vi "Frame Configuration Page.vi"(8 "error in (no error)":errorcluster, 11 "Node Ptr":T2 format="%.0x") -> (0 "error out":errorcluster)   [LabVIEW 2015, in "Protection and Rolling Counter Addon System Explorer.lvlib"]
uses:
  Protection and Rolling Counter Addon System Explorer.lvlib
  <vilib>/NI Veristand/Custom Device API/Custom Device Item Ref.ctl
  Shared/Types/Protection Type.ctl
  <vilib>/NI Veristand/Custom Device API/Custom Device API.lvlib
  Shared/Protection and Rolling Counter Addon Shared.lvlib
panel:
  in  "Protection Type":T1
  out "Frame ID":u32 format="%.0x"
  in  "Max Count":dbl=4.0
  out "Frame Rate":dbl
  out "Rolling Counter Channel":string
  out "CRC Channel":string
  in  "SHDocVw.IWebBrowser":refnum<k7>(container)
  in  "Value":dbl
  in  "Monitored Channels":i32(listbox)
  in  "Header":cluster{"Section Name":string}={"Section Name"="Custom Device Item Settings"}
  in  "Description":string
  in  "Name":string
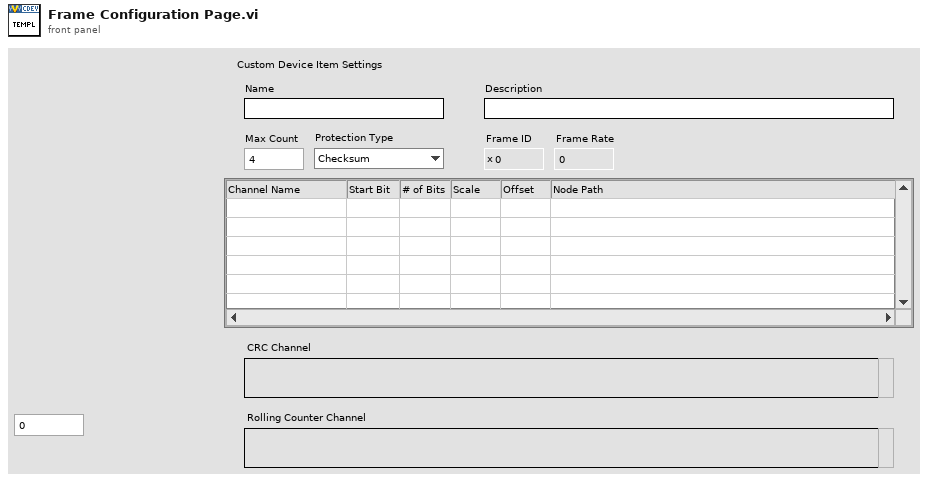
[diagram p1: front panel]
types:
  T1 = typedef "Protection and Rolling Counter Addon Shared.lvlib/Protection Type.ctl" = enum16{"Checksum", "CRC", "None (Counter Only)"}
  T2 = typedef "Custom Device API.lvlib/Custom Device Item Ref.ctl" = u64
  T3 = typedef "Custom Device API.lvlib/Custom Device Item Info.ctl" = cluster{"Name":string, "Is Channel":bool, "GUID":string, "Is Waveform":bool}
  T4 = typedef "Protection and Rolling Counter Addon Shared.lvlib/FrameConfiguration.ctl" = cluster{"Input Channels":T5[], "Frame Rate":dbl, "Rolling Counter Count":dbl, "PCL Count":u64, "Max Count":dbl, "Frame ID":u32, "Rolling Counter":T5, "CRC":T5, "Frame Name":string, "Cluster":string, "Database":string, "Protection Type":T1}
  T5 = typedef "Protection and Rolling Counter Addon Shared.lvlib/InputChannelConfiguration.ctl" = cluster{"Start Bit":i32, "Name":string, "Node Path":string, "Number of bits":i32, "Scale":dbl, "Offset":dbl, "Data Type":u32}
  T6 = typedef "Custom Device API.lvlib/Custom Device Commands.ctl" = enum16{"Default", "Item renamed", "Shutdown", "Dynamic button pressed"}
  T7 = typedef "LVPoint32TypeDef.ctl" = cluster{"Horizontal":i32, "Vertical":i32}
  T8 = typedef "LVRowAndColumnTypeDef.ctl" = cluster{"Row":i32, "Column":i32}
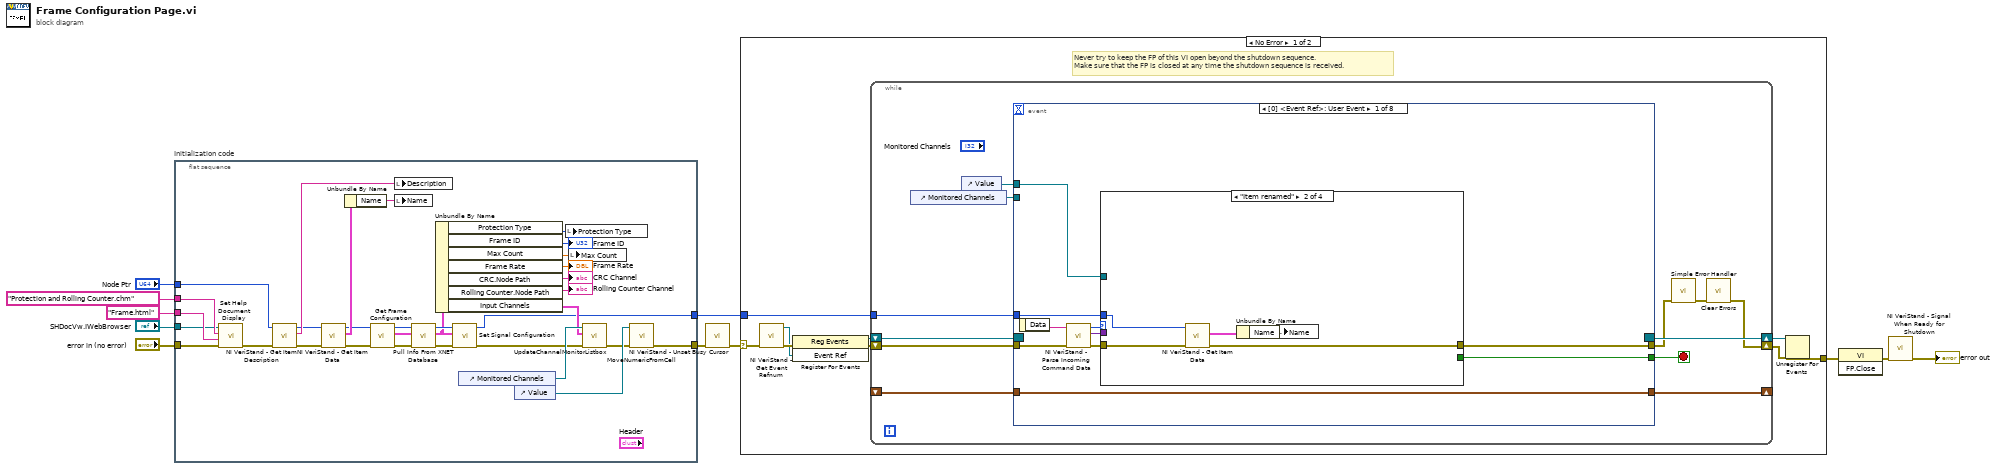
[diagram p0: block diagram]
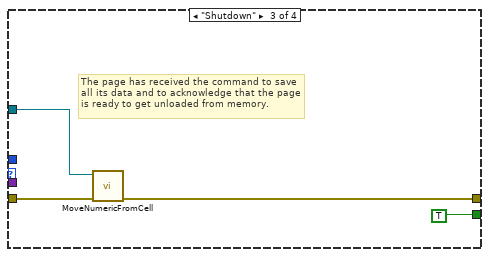
[diagram p3: hidden frame]
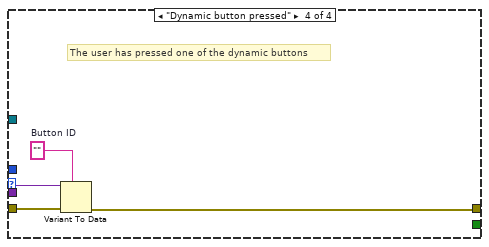
[diagram p4: hidden frame]
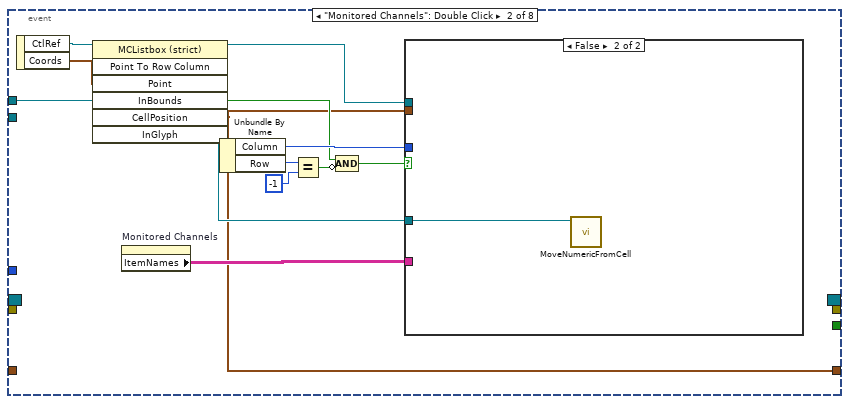
[diagram p5: hidden frame]
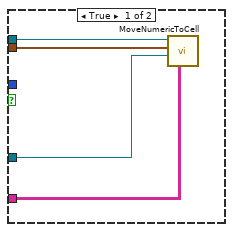
[diagram p6: hidden frame]
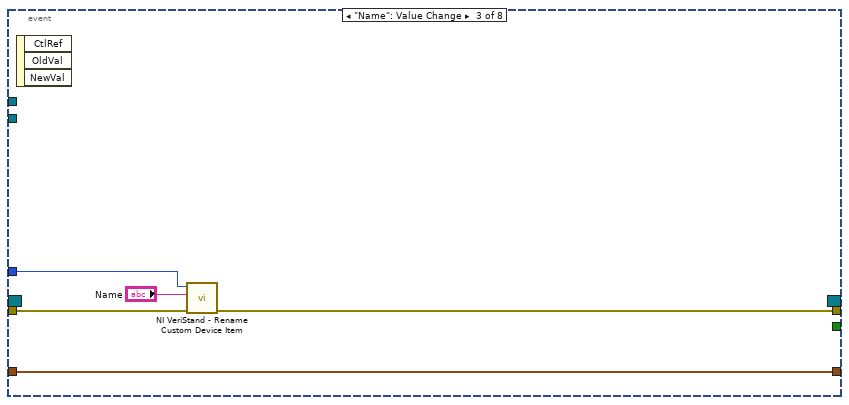
[diagram p7: hidden frame]
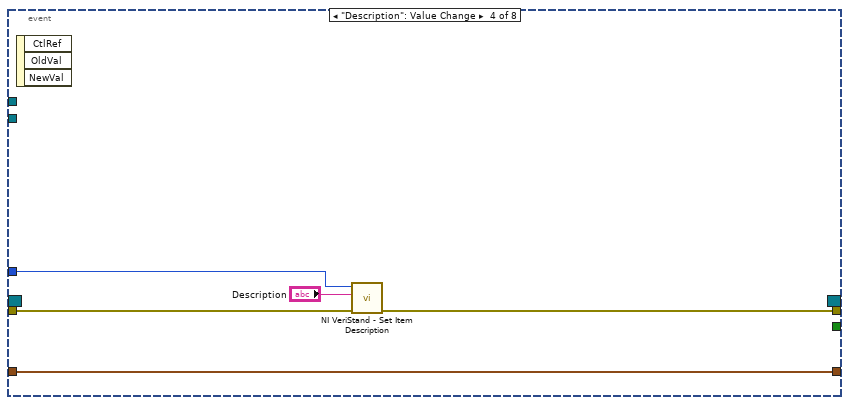
[diagram p8: hidden frame]
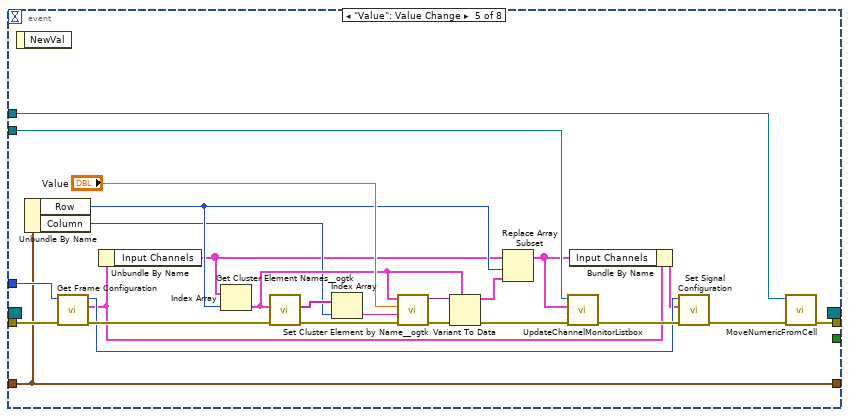
[diagram p9: hidden frame]
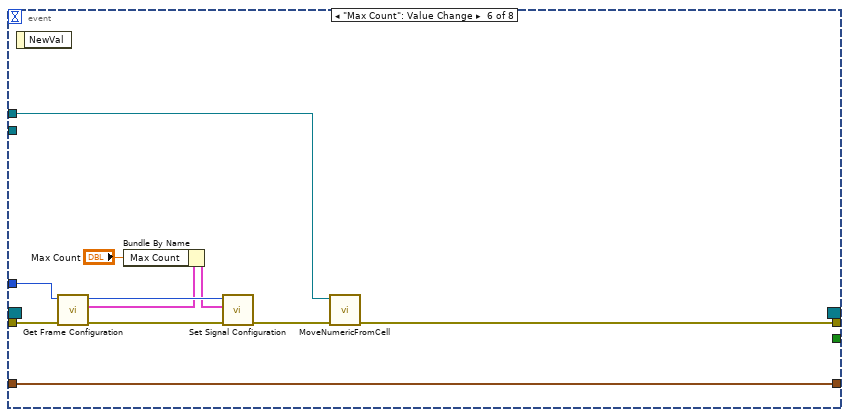
[diagram p10: hidden frame]
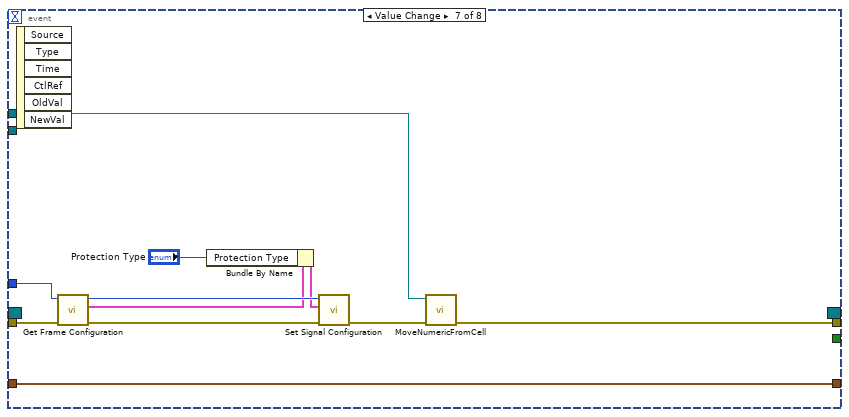
[diagram p11: hidden frame]
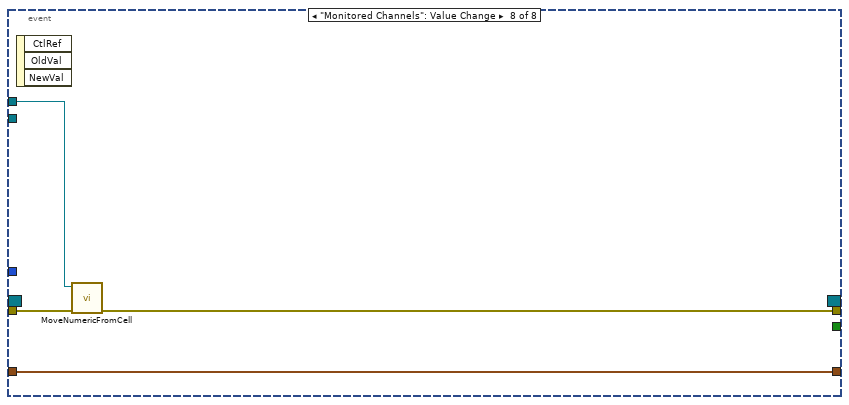
[diagram p12: hidden frame]
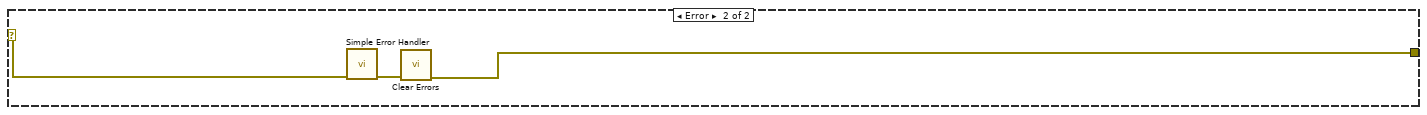
[diagram p13: hidden frame]
diagram:
  n1 = flat-sequence "Initialization code" {
    tunnel: "error in (no error)" -> [w39]
    tunnel: "Node Ptr" -> [w28]
    tunnel: [w36] -> w9
    tunnel: [w13] -> w7
    tunnel: "Protection and Rolling Counter.chm" ("Main CHM File") -> [w43]
    tunnel: "Frame.html" ("HTML File") -> [w42]
    tunnel: "SHDocVw.IWebBrowser" -> [w41]
    frame #0 {
      n2 = call "Set Help Document Display.vi"("error in (no error)"=w39, "HTML File"=w42, "Main CHM File"=w43, "SHDocVw.IWebBrowser2"=w41) -> ("error out"=w29:errorcluster)  [unwired: 7 in]
      n3 = call <vilib>:"NI VeriStand - Get Item Description.vi"("error in (no error)"=w29, "Item Ref in"=w28) -> ("error out"=w32:errorcluster, "Description"=w31:string, "Item Ref out"=w30:T2)  [unwired: 7 out]
      n4 = call <vilib>:"NI VeriStand - Get Item Data.vi"("error in (no error)"=w32, "Item Ref in"=w30) -> ("error out"=w19:errorcluster, "Item Info"=w33:T3, "Item Ref out"=w18:T2)  [unwired: 7 out]
      n5 = Unbundle By Name(w33) -> ("Name"=w34:string)
      n6 = call "Get Frame Configuration.vi"("error in"=w19, "Parent Ref"=w18) -> ("error out"=w20:errorcluster, "Selected Channels"=w16:T4, "Parent Ref Out"=w17:T2)  [unwired: 7 in]
      n7 = local write "Description"(w31) -> ()
      n8 = local write "Name"(w34) -> ()
      n9 = call "Pull Info From XNET Database.vi"("error in"=w20, "Frame Configuration"=w16, "Parent Ref"=w17) -> ("error out"=w21:errorcluster, "Frame Configuration"=w14:T4, "Item Ref out"=w15:T2)  [unwired: 6 in]
      n10 = Unbundle By Name(w14) -> ("Protection Type"=w22:T1, "Frame ID"=→"Frame ID":u32, "Max Count"=w24:dbl, "Frame Rate"=→"Frame Rate":dbl, "CRC.Node Path"=→"CRC Channel":string, "Rolling Counter.Node Path"=→"Rolling Counter Channel":string, "Input Channels"=w35:T5[])
      n11 = call "Set Signal Configuration.vi"("error in"=w21, "Selected Channels"=w14, "Parent Ref"=w15) -> ("error out"=w12:errorcluster, "Parent Ref Out"=w13:T2)  [unwired: 7 in]
      n12 = control-ref of="Monitored Channels"() -> (w40:refnum<vi>)
      n13 = control-ref of="Value"() -> (w38:refnum<vi>)
      n14 = local write "Protection Type"(w22) -> ()
      n15 = local write "Max Count"(w24) -> ()
      n16 = call "UpdateChannelMonitorListbox.vi"("error in (no error)"=w12, "Monitored Channels"=w35, "Listbox"=w40) -> ("error out"=w37:errorcluster)  [unwired: 8 in]
      n17 = call "MoveNumericFromCell.vi"("error in (no error)"=w37, "Digital in"=w38) -> ("error out"=w36:errorcluster)  [unwired: 9 in]
    }
  }
  n18 = call <vilib>:"NI VeriStand - Unset Busy Cursor.vi"("error in (no error)"=w9) -> ("error out"=w8:errorcluster)  [unwired: 10 out]
  n19 = case shown="No Error" w8 {
    selector: w8 -> [w44 w169]
    tunnel: [w49 w167] -> w11
    tunnel: w7 -> [w45 _]
    frame No Error {
      # "Never try to keep the FP of this VI open beyond the shutdown sequence.\nMake sure that the FP is closed at any time the shutdown sequence is received."
      n20 = call <vilib>:"NI VeriStand - Get Event Refnum.vi"("error in (no error)"=w44) -> ("error out"=w52:errorcluster, "Event Ref"=w48:refnum<user-event>)  [unwired: 9 out]
      n21 = register-events(error in=w52, w48) -> (reference out=w46:refnum<event-registration>, error out=w47:errorcluster)  [unwired: 1 in]
      n22 = while {
        tunnel: w45 -> [w60]
        shift-right: [w57] -> w50
        shift-left: w47 -> [w63]
        shift-right: [w64] -> w51
        shift-left: w46 -> [w62]
        shift-right: [w55] -> _
        shift-left: _ -> [w54]
        stop <- w61 stop-if-true
        n23 = control-ref of="Monitored Channels"() -> (w53:refnum<vi>)
        n24 = control-ref of="Value"() -> (w56:refnum<vi>)
        n25 = event shown="[0] <Event Ref>: User Event" {
          selector: w62 -> [_ _ _ _ _ _ _ _]
          dyn-events: [_ _ _ _ _ _ _ _] -> w64
          timeout: _ -> [_ _ _ _ _ _ _ _]
          tunnel: w63 -> [w74 _ w108 w113 w138 w149 w160 w164]
          tunnel: [w70 _ _ _ _ _ _ _] -> w61
          tunnel: [w69 _ w106 w112 w122 w146 w157 w163] -> w59
          tunnel: w60 -> [w68 _ w107 w111 w139 w150 w161 _]
          tunnel: w56 -> [w65 w96 _ _ w140 w151 w162 w165]
          tunnel: [w66 w89 w110 w115 w134 w147 w158 w166] -> w55
          tunnel: w54 -> [w66 _ w110 w115 w134 w147 w158 w166]
          tunnel: w53 -> [_ _ _ _ w137 _ _ _]
          event User Event {
            n26 = event-data() -> ("Data"=w73:string)  [unwired: 1 out]
            n27 = call <vilib>:"NI VeriStand - Parse Incoming Command Data.vi"("error in (no error)"=w74, "Incoming data"=w73) -> ("error out"=w72:errorcluster, "Outgoing data"=w67:variant, "Action"=w71:T6)  [unwired: 7 out]
            n28 = case shown="\"Item renamed\"" w71 {
              tunnel: w72 -> [w75 w78 w82 w88]
              tunnel: [_ _ TRUE _] -> w70
              tunnel: [w75 w77 w81 w85] -> w69
              tunnel: w68 -> [_ w76 _ _]
              tunnel: w67 -> [_ _ _ w87]
              tunnel: w65 -> [_ _ w83 _]
              frame "Default", Default {
              }
              frame "Item renamed" {
                n29 = call <vilib>:"NI VeriStand - Get Item Data.vi"("error in (no error)"=w78, "Item Ref in"=w76) -> ("error out"=w77:errorcluster, "Item Info"=w79:T3)  [unwired: 8 out]
                n30 = Unbundle By Name(w79) -> ("Name"=w80:string)
                n31 = local write "Name"(w80) -> ()
              }
              frame "Shutdown" {
                # "The page has received the command to save all its data and to acknowledge that the page is ready to get unloaded from memory."
                n32 = call "MoveNumericFromCell.vi"("error in (no error)"=w82, "Digital in"=w83) -> ("error out"=w81:errorcluster)  [unwired: 9 in]
              }
              frame "Dynamic button pressed" {
                w86 = ""  # Button ID
                # "The user has pressed one of the dynamic buttons"
                n33 = Variant To Data(error in=w88, type=w86, Variant=w87) -> (error out=w85:errorcluster)  [unwired: 1 out]
              }
            }
          }
          event "Monitored Channels": Double Click {
            n34 = event-data() -> ("CtlRef"=w99:refnum<vi>, "Coords"=w98:T7)  [unwired: 1 out]
            n35 = invoke class="MCListbox (strict)" method="Point To Row Column"(reference=w99, "Point"=w98) -> (reference out=w97:refnum<vi>, "InBounds"=w93:bool, "CellPosition"=w89:T8)  [unwired: 5 in, 4 out]
            n36 = property on="Monitored Channels" class="MCListbox (strict)"() -> ("ItemNames"=w90:string[][])  [unwired: 2 in, 2 out]
            n37 = Unbundle By Name(w89) -> ("Column"=w100:i32, "Row"=w94:i32)
            n38 = Equal?(x=w94, y=-1) -> (x = y?=w92:bool)
            n39 = Compound Arithmetic op=AND(w93, invert w92) -> (w91:bool)
            n40 = case shown="False" w91 {
              tunnel: w100 -> [_ _]
              tunnel: w97 -> [w104 _]
              tunnel: w89 -> [w103 _]
              tunnel: w96 -> [w102 w105]
              tunnel: w90 -> [w101 _]
              frame True {
                n41 = call "MoveNumericToCell.vi"("Data"=w101, "Numeric"=w102, "Cell Position"=w103, "Listbox"=w104) -> ()  [unwired: 7 in, 1 out]
              }
              frame False {
                n42 = call "MoveNumericFromCell.vi"("Digital in"=w105) -> ()  [unwired: 10 in, 1 out]
              }
            }
          }
          event "Name": Value Change {
            n43 = event-data() -> ()  [unwired: 4 out]
            n44 = call <vilib>:"NI VeriStand - Rename Custom Device Item.vi"("error in (no error)"=w108, "New Name"="Name", "Item Ref in"=w107) -> ("error out"=w106:errorcluster)  [unwired: 1 in, 7 out]
          }
          event "Description": Value Change {
            n45 = event-data() -> ()  [unwired: 4 out]
            n46 = call <vilib>:"NI VeriStand - Set Item Description.vi"("error in (no error)"=w113, "Description"="Description", "Item Ref in"=w111) -> ("error out"=w112:errorcluster)  [unwired: 8 out]
          }
          event "Value": Value Change {
            n47 = event-data() -> ()  [unwired: 2 out]
            n48 = Unbundle By Name(w134) -> ("Row"=w123:i32, "Column"=w121:i32)
            n49 = call "Get Frame Configuration.vi"("error in"=w138, "Parent Ref"=w139) -> ("error out"=w127:errorcluster, "Selected Channels"=w118:T4, "Parent Ref Out"=w120:T2)  [unwired: 7 in]
            n50 = Unbundle By Name(w118) -> ("Input Channels"=w119:T5[])
            n51 = Index Array(array=w119, index=w123) -> (element=w125:T5)
            n52 = call <userlib>:"Get Cluster Element Names__ogtk.vi"("error in (no error)"=w127, "Cluster"=w125) -> ("error out"=w128:errorcluster, "Element Names"=w133:string[])  [unwired: 8 in]
            n53 = Index Array(array=w133, index=w121) -> (element=w132:string)
            n54 = call <userlib>:"Set Cluster Element by Name__ogtk.vi"("error in (no error)"=w128, "Element Name (\"\": New Element Data Name)"=w132, "New Element Value"="Value", "Cluster"=w125) -> ("error out"=w129:errorcluster, "VCluster out"=w130:variant)  [unwired: 5 in, 1 out]
            n55 = Variant To Data(error in=w129, type=w125, Variant=w130) -> (data=w124:T5, error out=w126:errorcluster)
            n56 = Replace Array Subset(array=w119, new element=w124, index=w123) -> (w117:T5[])
            n57 = call "UpdateChannelMonitorListbox.vi"("error in (no error)"=w126, "Monitored Channels"=w117, "Listbox"=w137) -> ("error out"=w136:errorcluster)  [unwired: 8 in]
            n58 = Bundle By Name(cluster=w118, "Input Channels"=w117) -> (w116:T4)
            n59 = call "Set Signal Configuration.vi"("error in"=w136, "Selected Channels"=w116, "Parent Ref"=w120) -> ("error out"=w135:errorcluster)  [unwired: 7 in, 1 out]
            n60 = call "MoveNumericFromCell.vi"("error in (no error)"=w135, "Digital in"=w140) -> ("error out"=w122:errorcluster)  [unwired: 9 in]
          }
          event "Max Count": Value Change {
            n61 = event-data() -> ()  [unwired: 2 out]
            n62 = call "Get Frame Configuration.vi"("error in"=w149, "Parent Ref"=w150) -> ("error out"=w142:errorcluster, "Selected Channels"=w144:T4, "Parent Ref Out"=w145:T2)  [unwired: 7 in]
            n63 = Bundle By Name(cluster=w144, "Max Count"="Max Count") -> (w143:T4)
            n64 = call "Set Signal Configuration.vi"("error in"=w142, "Selected Channels"=w143, "Parent Ref"=w145) -> ("error out"=w148:errorcluster)  [unwired: 7 in, 1 out]
            n65 = call "MoveNumericFromCell.vi"("error in (no error)"=w148, "Digital in"=w151) -> ("error out"=w146:errorcluster)  [unwired: 9 in]
          }
          event Value Change {
            n66 = event-data() -> ()  [unwired: 7 out]
            n67 = call "Get Frame Configuration.vi"("error in"=w160, "Parent Ref"=w161) -> ("error out"=w153:errorcluster, "Selected Channels"=w155:T4, "Parent Ref Out"=w156:T2)  [unwired: 7 in]
            n68 = Bundle By Name(cluster=w155, "Protection Type"="Protection Type") -> (w154:T4)
            n69 = call "Set Signal Configuration.vi"("error in"=w153, "Selected Channels"=w154, "Parent Ref"=w156) -> ("error out"=w159:errorcluster)  [unwired: 7 in, 1 out]
            n70 = call "MoveNumericFromCell.vi"("error in (no error)"=w159, "Digital in"=w162) -> ("error out"=w157:errorcluster)  [unwired: 9 in]
          }
          event "Monitored Channels": Value Change {
            n71 = event-data() -> ()  [unwired: 4 out]
            n72 = call "MoveNumericFromCell.vi"("error in (no error)"=w164, "Digital in"=w165) -> ("error out"=w163:errorcluster)  [unwired: 9 in]
          }
        }
        n73 = call <vilib>:"Simple Error Handler.vi"("error in (no error)"=w59) -> ("error out"=w58:errorcluster)  [unwired: 1 in, 7 out]
        n74 = call <vilib>:"Clear Errors.vi"("error in (no error)"=w58) -> ("error out"=w57:errorcluster)  [unwired: 1 in, 5 out]
      }
      n75 = Unregister For Events(event registration refnum=w51, error in=w50) -> (error out=w49:errorcluster)
    }
    frame Error {
      n76 = call <vilib>:"Simple Error Handler.vi"("error in (no error)"=w169) -> ("error out"=w168:errorcluster)  [unwired: 1 in, 7 out]
      n77 = call <vilib>:"Clear Errors.vi"("error in (no error)"=w168) -> ("error out"=w167:errorcluster)  [unwired: 1 in, 5 out]
    }
  }
  n78 = invoke class="VI" method="FP.Close"(error in=w11) -> (error out=w10:errorcluster)  [unwired: 2 in, 2 out]
  n79 = call <vilib>:"NI VeriStand - Signal When Ready for Shutdown.vi"("error in (no error)"=w10) -> ("error out"=→"error out":errorcluster)  [unwired: 10 out]
